vi "macro_SimpleMotorFF_Calculate.vi"   [LabVIEW 2019, in "Trajectory_Library.lvlib"]
uses:
  Trajectory_Library.lvlib
types:
  T1 = typedef "Trajectory_Library.lvlib/SIMPLE_MOTOR_FF.ctl" = cluster{"Ks":dbl, "Kv":dbl, "Ka":dbl, "KnInv":dbl}
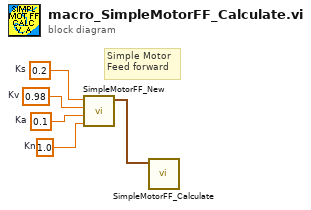
[diagram p0: block diagram]
diagram:
  w1 = 1.0  # Kn
  w2 = 0.2  # Ks
  w3 = 0.98  # Kv
  w4 = 0.1  # Ka
  # "Simple Motor\nFeed forward"
  n1 = call "SimpleMotorFF_New.vi"("Kn"=w1, "Ka"=w4, "Kv"=w3, "Ks"=w2) -> ("SIMPLE_MOTOR_FF"=w5:T1)  [unwired: 7 in]
  n2 = call "SimpleMotorFF_Calculate.vi"("SIMPLE_MOTOR_FF"=w5) -> ()  [unwired: 10 in, 1 out]
